vi "TMS Robot_adjust.vi"() -> ()   [LabVIEW 2018]
uses:
  <vilib>/Platform/TimedLoop/XDataNode/timing_clust.ctl
  <vilib>/Platform/TimedLoop/XDataNode/nitl_modes.ctl
  <vilib>/Platform/TimedLoop/XDataNode/wakeup.ctl
  <vilib>/myRIO/Instrument Drivers/Onboard IO/AI/typedefs/AI Reference.ctl
  <vilib>/myRIO/Common/Instrument Driver Framework/Utilities/typedefs/myRIO Generic Hardware Reference.ctl
  <vilib>/myRIO/Common/Instrument Driver Framework/Utilities/typedefs/Hardware Version Enum.ctl
  <vilib>/myRIO/Common/Instrument Driver Framework/Utilities/typedefs/myRIO v1.0 Reference.ctl
  <vilib>/myRIO/Common/Instrument Driver Framework/Utilities/typedefs/Generic FPGA Reference.ctl
  <vilib>/myRIO/Common/Instrument Driver Framework/myRIO v1.0/AI/typedefs/AI Channels List.ctl
  <vilib>/myRIO/Common/Instrument Driver Framework/myRIO v1.0/AI/typedefs/AI Channels Enum.ctl
  <vilib>/myRIO/Common/Instrument Driver Framework/Utilities/typedefs/Analog Scaling Constants List.ctl
  <vilib>/myRIO/Common/Instrument Driver Framework/Utilities/typedefs/Analog Scaling Constants.ctl
  <vilib>/userdefined/High Color/nirio_resource_hc.ctl
  <vilib>/myRIO/Instrument Drivers/Onboard IO/DIO/typedefs/DIO Reference.ctl
  <vilib>/myRIO/Common/Instrument Driver Framework/myRIO v1.0/DIO/typedefs/DIO Channels List.ctl
  <vilib>/myRIO/Common/Instrument Driver Framework/myRIO v1.0/DIO/typedefs/DIO Channels Enum.ctl
  <vilib>/myRIO/Common/Instrument Driver Framework/myRIO v1.0/AI/vis/myRIO v1.1 Open AI.vi
  <vilib>/myRIO/Common/Instrument Driver Framework/myRIO v1.0/DIO/vis/myRIO v1.1 Open DIO.vi
  <vilib>/myRIO/Common/Instrument Driver Framework/Utilities/vis/Validate Channels.vi
  <vilib>/myRIO/Common/Instrument Driver Framework/myRIO v1.0/AI/vis/myRIO v1.0 Reserve AI.vi
  <vilib>/myRIO/Common/Instrument Driver Framework/myRIO v1.0/DIO/vis/myRIO v1.0 Reserve DIO.vi
  <vilib>/myRIO/Common/Instrument Driver Framework/myRIO v1.0/DIO/vis/myRIO v1.0 Close DIO.vi
  <vilib>/myRIO/Common/Instrument Driver Framework/myRIO v1.0/AI/vis/myRIO v1.0 Build MUX Configuration AI.vi
  <vilib>/myRIO/Common/Instrument Driver Framework/myRIO v1.0/Resource Manager/vis/myRIO v1.0 Reserve Channel List.vi
  <vilib>/myRIO/Common/Instrument Driver Framework/myRIO v1.0/DIO/vis/myRIO v1.0 Build MUX Configuration DIO.vi
  <vilib>/myRIO/Common/Instrument Driver Framework/myRIO v1.0/DIO/vis/myRIO v1.0 Unreserve DIO.vi
  <vilib>/myRIO/Common/Instrument Driver Framework/myRIO v1.0/Resource Manager/vis/myRIO v1.0 Reserve Channel.vi
  <vilib>/myRIO/Common/Instrument Driver Framework/myRIO v1.0/Resource Manager/vis/myRIO v1.0 Unreserve Channel.vi
  <vilib>/myRIO/Common/Instrument Driver Framework/myRIO v1.0/Resource Manager/vis/myRIO v1.0 Create Configuration List.vi
  <vilib>/myRIO/Common/Instrument Driver Framework/myRIO v1.0/Resource Manager/vis/myRIO v1.0 Unreserve Channel List.vi
  <vilib>/myRIO/Common/Instrument Driver Framework/myRIO v1.0/Resource Manager/vis/myRIO v1.0 Build Mutex Name.vi
  <vilib>/Utility/VariantDataType/GetNumericInfo.vi
  <vilib>/Utility/error.llb/Error Cluster From Error Code.vi
  <vilib>/myRIO/Common/Instrument Driver Framework/myRIO v1.0/myRIO v1.1 Open.vi
  <vilib>/myRIO/Common/Instrument Driver Framework/Utilities/vis/IO Manager.vi
  <vilib>/myRIO/Common/Instrument Driver Framework/Utilities/vis/Configuration Manager.vi
  <vilib>/myRIO/Common/Instrument Driver Framework/myRIO v1.0/Resource Manager/vis/myRIO v1.0 Configure IO.vi
  <vilib>/myRIO/Common/Instrument Driver Framework/myRIO v1.0/myRIO v1.0 Close.vi
  <vilib>/myRIO/Common/Instrument Driver Framework/myRIO v1.0/AI/vis/myRIO v1.0 Get Scaling Constants AI.vi
  <vilib>/myRIO/Common/Instrument Driver Framework/myRIO v1.0/AI/vis/myRIO v1.0 Read AI.vi
  <vilib>/myRIO/Common/Instrument Driver Framework/myRIO v1.0/DIO/vis/myRIO v1.0 Write DIO.vi
  <vilib>/myRIO/Common/Instrument Driver Framework/myRIO v1.0/DIO/vis/myRIO v1.0 Shutdown DIO.vi
  <vilib>/Platform/TimedLoop/XDataNode/XDataNode.xnode
  <vilib>/myRIO/Instrument Drivers/Onboard IO/DIO/vis/myRIO DIO Open.xnode
  <vilib>/myRIO/Instrument Drivers/Onboard IO/AI/vis/myRIO AI Open.xnode
  <vilib>/Platform/TimedLoop/XDataNode/XDNodeRunTimeDep.lvlib
  <vilib>/myRIO/Instrument Drivers/Onboard IO/DIO/DIO.lvlib
  <vilib>/myRIO/Instrument Drivers/Onboard IO/AI/AI.lvlib
panel:
  out "Phi Real Output  TCP":dbl
  out "Theta Real Output TCP":dbl
  out "Curve Moving TCP":i16
  out "Psi Real Output TCP":dbl
  out "Psi Moving TCP":i16
  out "Z Real Output TCP":dbl
  out "Z Moving TCP":i16
  out "Y Real Output TCP":dbl
  out "Y Moving TCP":i16
  out "X Real Output TCP":dbl
  out "X Moving TCP":i16
  out "Optical R":dbl
  out "Optical L":dbl
  out "Optical psi":dbl
  out "Optical Z":dbl
  out "Optical Y":dbl
  out "Optical X":dbl
  in  "Stop number L":dbl
  in  "Stop number R":dbl
  in  "Stop number x":dbl
  in  "Stop number y":dbl
  in  "Stop number z":dbl
  in  "Stop number psi":dbl
  out "up L":bool
  out "left L":bool
  in  "Step/s  curve":dbl=4.0
  in  "Step difference L":dbl
  in  "Tab Control":enum32{"Azimuth", "Elevation"}(tab)
  in  "Right":bool
  in  "Left":bool
  out "Real Output theta":dbl
  in  "User Input theta":dbl
  in  "Up":bool
  in  "Down":bool
  out "Real Output Phi":dbl
  in  "User Input Phi":dbl=10.45218049
  in  "Motor Input L":dbl
  out "down L":bool
  out "right L":bool
  out "Moving":bool
  out "up R":bool
  out "left R":bool
  in  "Step difference R":dbl
  in  "Motor Input R":dbl
  out "down R":bool
  out "right R":bool
  out "Moving R":bool
  out "up z":bool
  out "down z":bool
  out "right z":bool
  out "left z":bool
  in  "Step/s z":dbl=4.0
  out "Motor Position z":dbl
  in  "User Input z":dbl
  out "Motor State z":dbl
  out "Real Output z":dbl
  in  "Step diff z":dbl
  in  "Up z":bool
  in  "Motor Input z":dbl
  in  "Down z":bool
  out "Moving z":bool
  out "up x":bool
  out "down x":bool
  out "right x":bool
  out "left x":bool
  in  "Step/s x":dbl=4.0
  out "Motor Position x":dbl
  in  "User Input x":dbl
  out "Motor State x":dbl
  out "Real Output x":dbl
  in  "Step diff x":dbl
  in  "Forward x":bool
  in  "Motor Input x":dbl
  in  "Backward x":bool
  out "Moving x":bool
  out "up y":bool
  out "down y":bool
  out "right y":bool
  out "left y":bool
  in  "Step/s y":dbl=4.0
  out "Motor Position y":dbl
  in  "User Input y":dbl
  out "Motor State y":dbl
  out "Real Output y":dbl
  in  "Step diff y":dbl
  in  "Left y":bool
  in  "Motor Input y":dbl
  in  "Right y":bool
  out "Moving y":bool
  out "up psi":bool
  out "down psi":bool
  out "right psi":bool
  out "left psi":bool
  in  "Step/s psi":dbl=4.0
  out "Motor Position psi":dbl
  in  "User Input psi":dbl
  out "Motor State psi":dbl
  out "Real Output psi":dbl
  in  "Step diff psi":dbl
  in  "Left psi":bool
  in  "Motor Input psi":dbl
  in  "Right psi":bool
  out "Moving psi":bool
  in  "Stop":bool
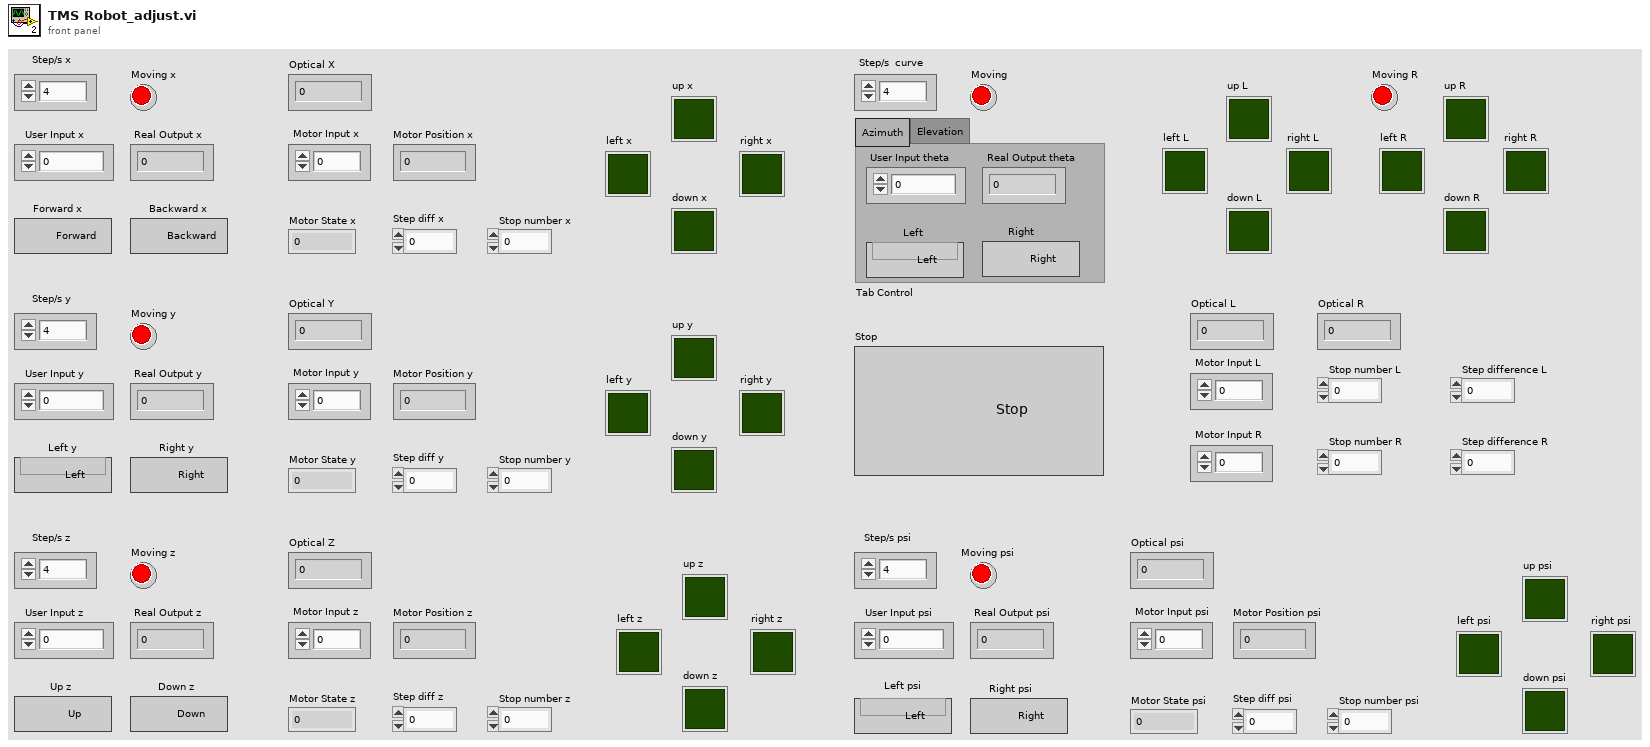
[diagram p1: front panel]
types:
  T1 = enum16{"big-endian, network order", "native, host order", "little-endian"}
  T2 = typedef "nirio_resource_hc.ctl" = tag
  T3 = typedef "Hardware Version Enum.ctl" = enum16{"Unknown", "myRIO-1900", "myRIO-1950", "roboRIO", "NI ELVIS RIO CM", "ELVIS III"}
  T4 = typedef "XDNodeRunTimeDep.lvlib/timing_clust.ctl" = cluster{"Expected End [f-1]":u64, "Actual End [f-1]":u64, "Finished Late? [f-1]":bool, "Expected End [i-1]":u64, "Actual End [i-1]":u64, "Finished Late? [i-1]":bool, "Expected Start [i]":u64, "Actual Start [i]":u64, "Expected Start [f]":u64, "Actual Start [f]":u64, "Source Name":string, "Structure Name":string, "Period":i64, "Deadline":i64, "Offset":i64, "Start":i64, "Priority":i32, "Timeout":i32, "Mode":T5, "Wakeup Reason":T6, "Error":errorcluster, "Source Type":string, "Secondary Source Type":string, "Global End Time":u64, "Global Start Time":u64, "Frame Duration":u64, "Iteration Duration":u64, "Assigned CPU":i32, "I/O Scan Engine Mode":u32}
  T5 = typedef "XDNodeRunTimeDep.lvlib/nitl_modes.ctl" = enum32{"No Change", "Process missed periods, maintain original phase", "Discard missed periods, maintain original phase", "Process missed periods, ignore original phase", "Discard missed periods, ignore original phase"}
  T6 = typedef "XDNodeRunTimeDep.lvlib/wakeup.ctl" = enum32{"Normal", "Aborted", "Asynchronous wakeup", "Timing source error", "Timed loop error", "Timeout"}
  T7 = typedef "AI.lvlib/AI Reference.ctl" = cluster{"myRIO Reference":T8, "AI Channels List":T11, "AI Scaling Constants List":T13}
  T8 = typedef "myRIO Generic Hardware Reference.ctl" = cluster{"myRIO Model":T3, "myRIO Hardware Reference":T9}
  T9 = typedef "myRIO v1.0 Reference.ctl" = cluster{"Generic FPGA Reference":T10, "Allow multiple opens":bool}
  T10 = typedef "Generic FPGA Reference.ctl" = refnum<k20>
  T11 = typedef "AI Channels List.ctl" = T12[]
  T12 = typedef "AI Channels Enum.ctl" = enum16{"Not Connected", "AudioIn/Left", "AudioIn/Right", "C/AI0", "C/AI1", "A/AI0", "A/AI1", "A/AI2", "A/AI3", "A/AI4", "A/AI5", "A/AI6", "A/AI7", "B/AI0", "B/AI1", "B/AI2", "B/AI3", "B/AI4", "B/AI5", "B/AI6", "B/AI7", "AI/AI0", "AI/AI1", "AI/AI2", "AI/AI3", "A/AI0 (DIFF)", "A/AI1 (DIFF)", "A/AI2 (DIFF)", "A/AI3 (DIFF)", "B/AI0 (DIFF)", "B/AI1 (DIFF)", "B/AI2 (DIFF)", "B/AI3 (DIFF)"}
  T13 = typedef "Analog Scaling Constants List.ctl" = T14[]
  T14 = typedef "Analog Scaling Constants.ctl" = cluster{"LSB Weight (Volts)":dbl, "Offset (Volts)":dbl, "Signed?":bool}
  T15 = typedef "DIO.lvlib/DIO Reference.ctl" = cluster{"myRIO Reference":T8, "DIO Channels List":T16}
  T16 = typedef "DIO Channels List.ctl" = T17[]
  T17 = typedef "DIO Channels Enum.ctl" = enum16{"Not Connected", "C/DIO0", "C/DIO1", "C/DIO2", "C/DIO3", "C/DIO4", "C/DIO5", "C/DIO6", "C/DIO7", "A/DIO0", "A/DIO1", "A/DIO2", "A/DIO3", "A/DIO4", "A/DIO5", "A/DIO6", "A/DIO7", "A/DIO8", "A/DIO9", "A/DIO10", "A/DIO11", "A/DIO12", "A/DIO13", "A/DIO14", "A/DIO15", "A/DIO16", "A/DIO17", "A/DIO18", "A/DIO19", "B/DIO0", "B/DIO1", "B/DIO2", "B/DIO3", "B/DIO4", "B/DIO5", "B/DIO6", "B/DIO7", "B/DIO8", "B/DIO9", "B/DIO10", "B/DIO11", "B/DIO12", "B/DIO13", "B/DIO14", "B/DIO15", "B/DIO16", "B/DIO17", "B/DIO18", "B/DIO19", "LED0", "LED1", "LED2", "LED3", "Button0", "DIO/DIO0", "DIO/DIO1", "DIO/DIO2", "DIO/DIO3", "DIO/DIO4", "DIO/DIO5", "DIO/DIO6", "DIO/DIO7", "DIO/DIO8", "DIO/DIO9", "SPI/CS0", "SPI/CS1", "SPI/CS2", "SPI/CS3", "LED RADIO (Green)", "LED RADIO (Red)", "LED COMM (Green)", "LED COMM (Red)", "LED MODE (Green)", "LED MODE (Red)"}
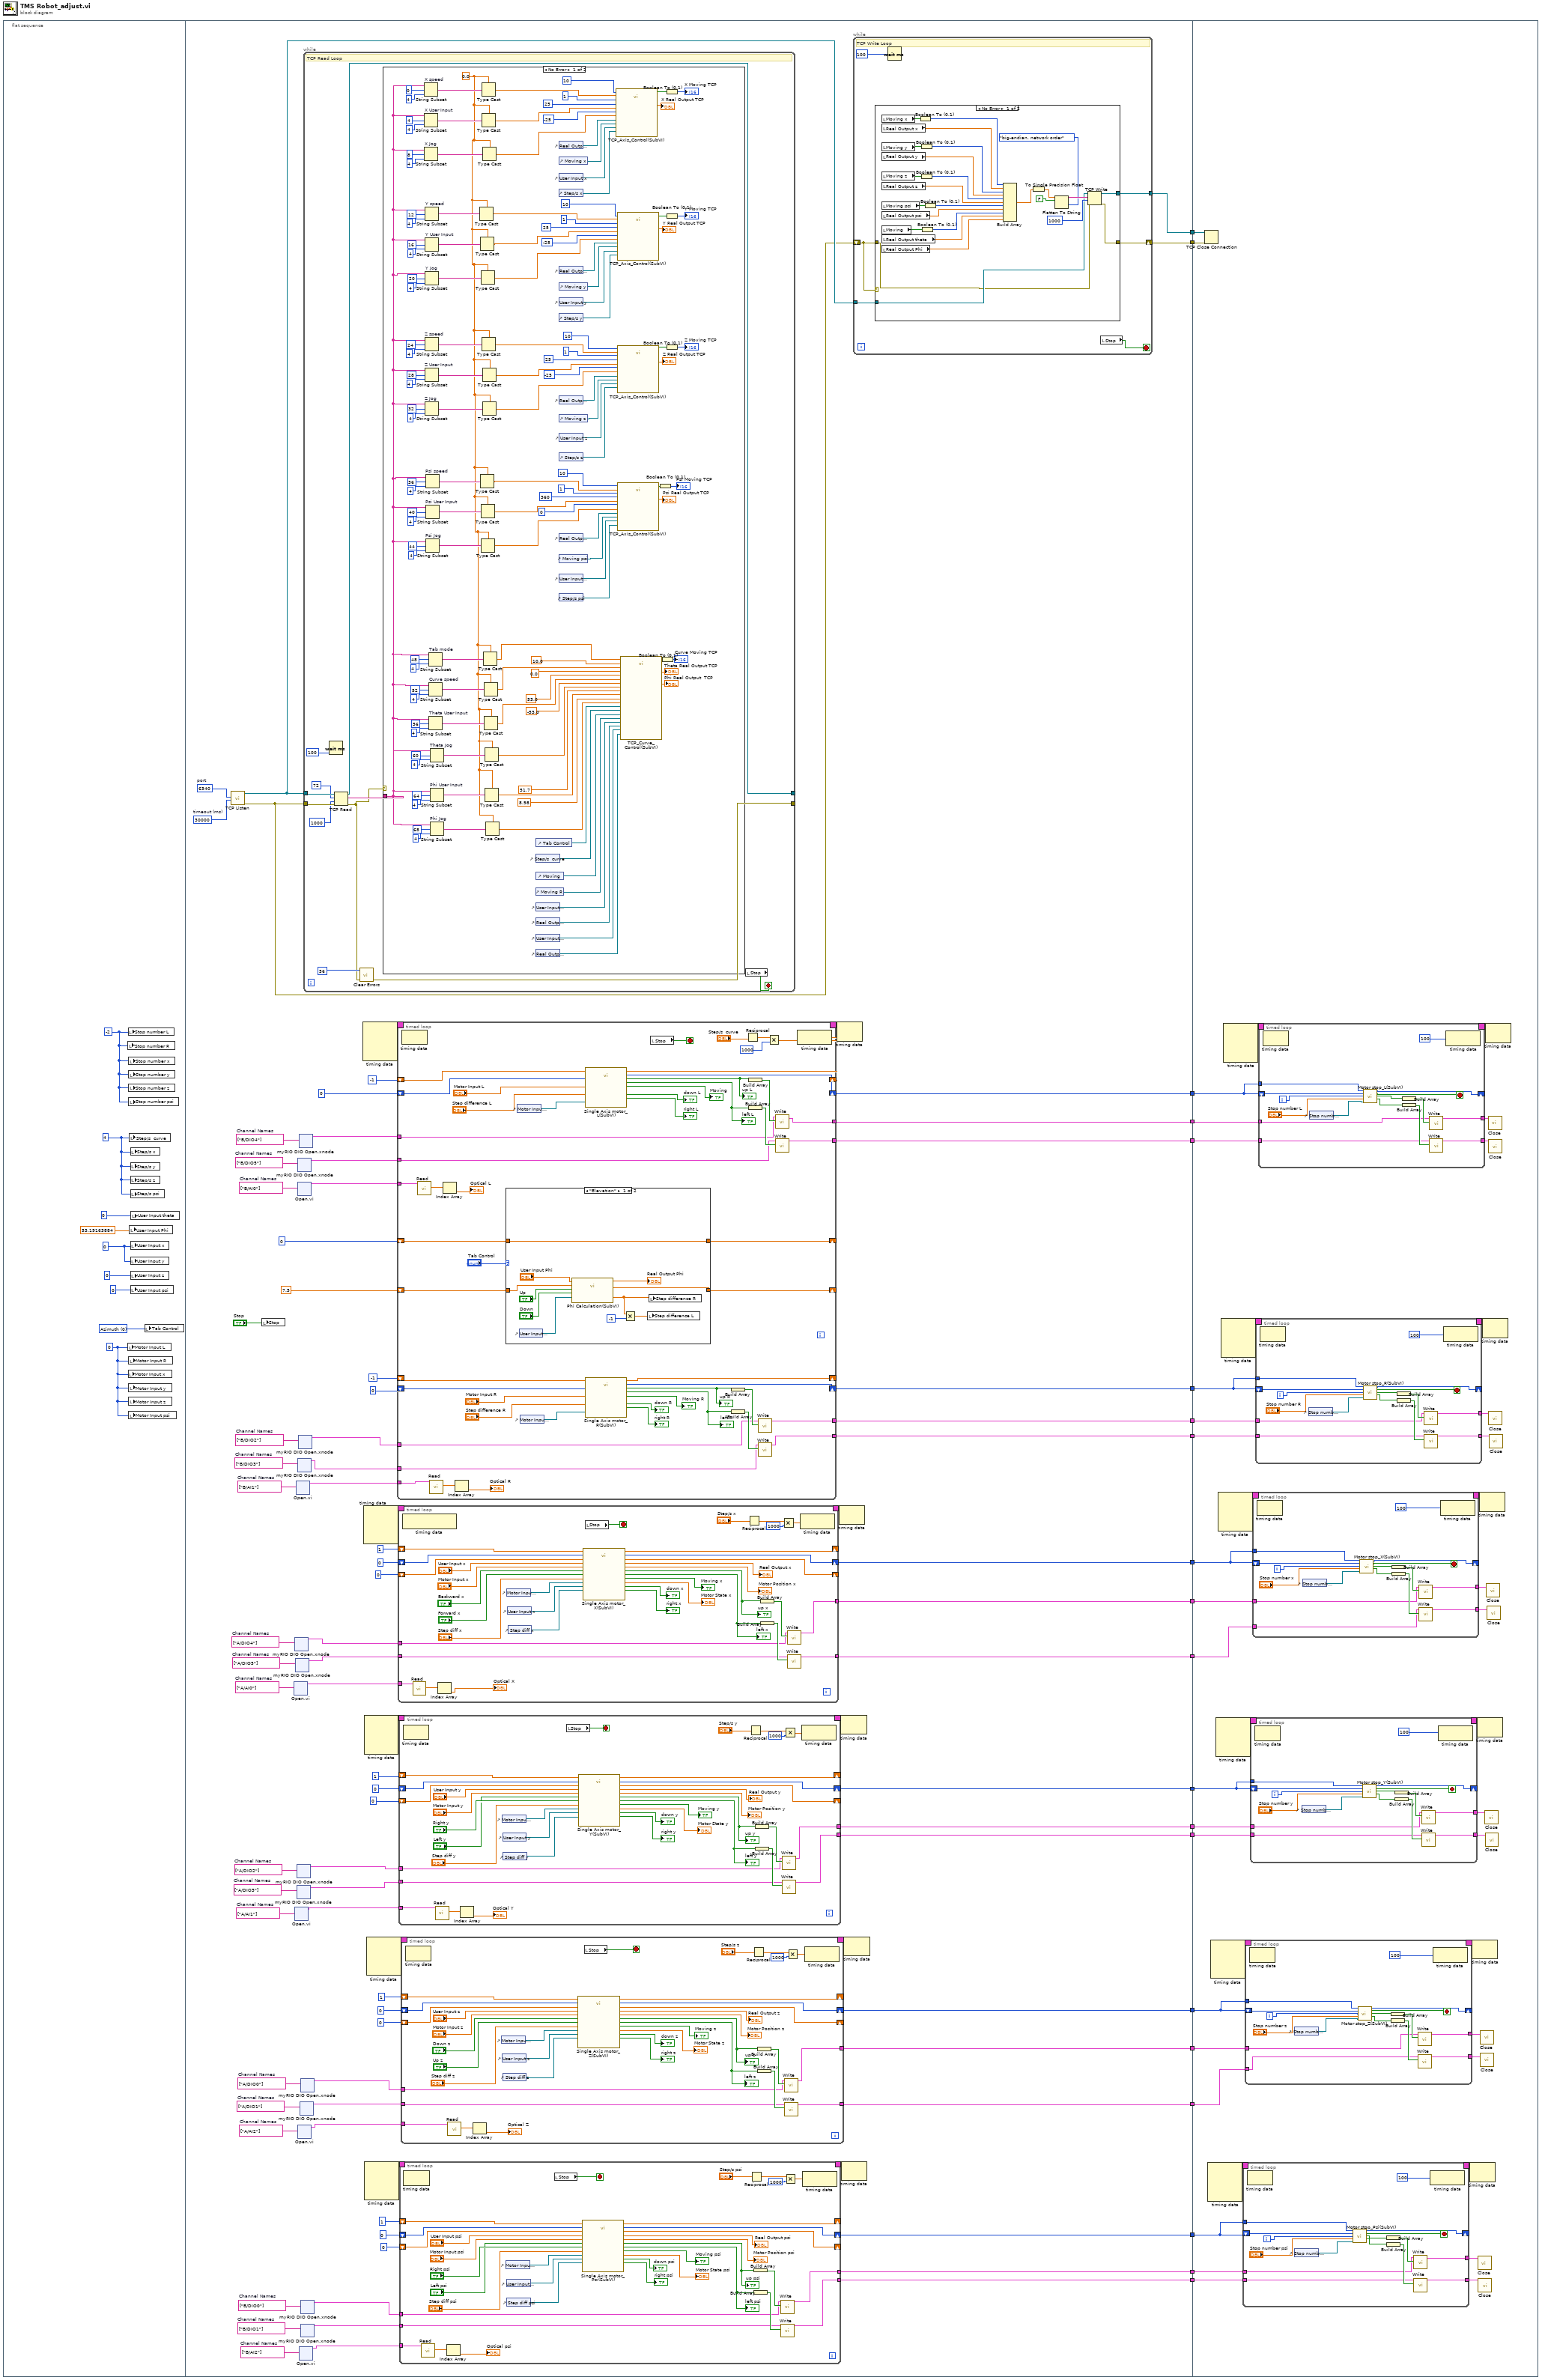
[diagram p0: block diagram]
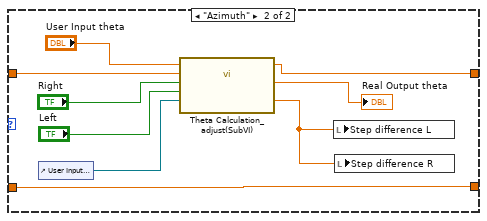
[diagram p4: hidden frame]
diagram:
  n1 = flat-sequence {
    tunnel: [w96] -> w20
    tunnel: [w95] -> w19
    tunnel: [w94] -> w18
    tunnel: [w93] -> w17
    tunnel: [w92] -> w16
    tunnel: [w91] -> w15
    tunnel: [w90] -> w14
    tunnel: [w89] -> w13
    tunnel: [w88] -> w12
    tunnel: [w87] -> w11
    tunnel: [w86] -> w10
    tunnel: [w85] -> w9
    tunnel: [w84] -> w8
    tunnel: [w83] -> w7
    tunnel: [w82] -> w6
    tunnel: [w81] -> w5
    tunnel: [w80] -> w4
    tunnel: [w79] -> w3
    tunnel: [w33] -> w2
    tunnel: [w32] -> w1
    tunnel: w20 -> [w887]
    tunnel: w19 -> [w884]
    tunnel: w18 -> [w881]
    tunnel: w17 -> [w878]
    tunnel: w16 -> [w875]
    tunnel: w15 -> [w872]
    tunnel: w14 -> [w869]
    tunnel: w13 -> [w868]
    tunnel: w12 -> [w867]
    tunnel: w11 -> [w866]
    tunnel: w10 -> [w861]
    tunnel: w9 -> [w860]
    tunnel: w8 -> [w859]
    tunnel: w7 -> [w858]
    tunnel: w6 -> [w857]
    tunnel: w5 -> [w856]
    tunnel: w4 -> [w855]
    tunnel: w3 -> [w854]
    tunnel: w2 -> [w847]
    tunnel: w1 -> [w846]
    frame #0 {
      w21 = 0
      w22 = u16 0 items=["Azimuth"]
      w24 = 0
      w28 = -2
      w27 = 4
      n2 = local write "Stop number R"(w28) -> ()
      n3 = local write "Motor Input L"(w21) -> ()
      n4 = local write "Stop number L"(w28) -> ()
      n5 = local write "Motor Input x"(w21) -> ()
      n6 = local write "Stop number x"(w28) -> ()
      n7 = local write "Stop number y"(w28) -> ()
      n8 = local write "Stop number z"(w28) -> ()
      n9 = local write "Stop number psi"(w28) -> ()
      n10 = local write "Motor Input R"(w21) -> ()
      n11 = local write "Motor Input y"(w21) -> ()
      n12 = local write "Motor Input z"(w21) -> ()
      n13 = local write "Motor Input psi"(w21) -> ()
      n14 = local write "Step/s  curve"(w27) -> ()
      n15 = local write "User Input Phi"(53.19163884) -> ()
      n16 = local write "Step/s x"(w27) -> ()
      n17 = local write "Step/s y"(w27) -> ()
      n18 = local write "Step/s z"(w27) -> ()
      n19 = local write "Step/s psi"(w27) -> ()
      n20 = local write "User Input x"(w24) -> ()
      n21 = local write "User Input y"(w24) -> ()
      n22 = local write "User Input z"(0) -> ()
      n23 = local write "User Input psi"(0) -> ()
      n24 = local write "User Input theta"(0) -> ()
      n25 = local write "Tab Control"(w22) -> ()
    }
    frame #1 {
      w34 = u16 6340  # port
      w35 = 30000  # timeout (ms)
      w44 = tag[] ["B/AI0"]  # Channel Names
      w46 = tag[] ["B/AI1"]  # Channel Names
      w49 = tag[] ["B/AI2"]  # Channel Names
      w51 = tag[] ["A/AI2"]  # Channel Names
      w53 = tag[] ["A/AI1"]  # Channel Names
      w55 = tag[] ["A/AI0"]  # Channel Names
      w59 = tag[] ["B/DIO1"]  # Channel Names
      w58 = tag[] ["B/DIO0"]  # Channel Names
      w63 = tag[] ["A/DIO1"]  # Channel Names
      w62 = tag[] ["A/DIO0"]  # Channel Names
      w67 = tag[] ["A/DIO3"]  # Channel Names
      w66 = tag[] ["A/DIO2"]  # Channel Names
      w71 = tag[] ["A/DIO5"]  # Channel Names
      w70 = tag[] ["A/DIO4"]  # Channel Names
      w75 = tag[] ["B/DIO5"]  # Channel Names
      w74 = tag[] ["B/DIO4"]  # Channel Names
      w78 = tag[] ["B/DIO3"]  # Channel Names
      w77 = tag[] ["B/DIO2"]  # Channel Names
      n26 = call <vilib>:"TCP Listen.vi"("timeout ms (wait forever: -1)"=w35, "port"=w34) -> ("error out"=w30:errorcluster, "connection ID"=w31:refnum<k5>)  [unwired: 5 in, 3 out]
      n27 = local write "Stop"("Stop") -> ()
      n28 = xnode "Open.vi"("Channel Names"=w55) -> ("AI Ref Out"=w54:T7)  [unwired: 2 in, 1 out]
      n29 = xnode "myRIO DIO Open.xnode"("Channel Names"=w70) -> ("DIO Ref Out"=w69:T15)  [unwired: 2 in, 1 out]
      n30 = xnode "Open.vi"("Channel Names"=w53) -> ("AI Ref Out"=w52:T7)  [unwired: 2 in, 1 out]
      n31 = xnode "myRIO DIO Open.xnode"("Channel Names"=w71) -> ("DIO Ref Out"=w68:T15)  [unwired: 2 in, 1 out]
      n32 = xnode "Open.vi"("Channel Names"=w46) -> ("AI Ref Out"=w45:T7)  [unwired: 2 in, 1 out]
      n33 = xnode "myRIO DIO Open.xnode"("Channel Names"=w67) -> ("DIO Ref Out"=w64:T15)  [unwired: 2 in, 1 out]
      n34 = xnode "myRIO DIO Open.xnode"("Channel Names"=w66) -> ("DIO Ref Out"=w65:T15)  [unwired: 2 in, 1 out]
      n35 = xnode "myRIO DIO Open.xnode"("Channel Names"=w75) -> ("DIO Ref Out"=w72:T15)  [unwired: 2 in, 1 out]
      n36 = xnode "Open.vi"("Channel Names"=w44) -> ("AI Ref Out"=w43:T7)  [unwired: 2 in, 1 out]
      n37 = xnode "myRIO DIO Open.xnode"("Channel Names"=w78) -> ("DIO Ref Out"=w47:T15)  [unwired: 2 in, 1 out]
      n38 = xnode "Open.vi"("Channel Names"=w51) -> ("AI Ref Out"=w50:T7)  [unwired: 2 in, 1 out]
      n39 = xnode "myRIO DIO Open.xnode"("Channel Names"=w77) -> ("DIO Ref Out"=w76:T15)  [unwired: 2 in, 1 out]
      n40 = xnode "myRIO DIO Open.xnode"("Channel Names"=w74) -> ("DIO Ref Out"=w73:T15)  [unwired: 2 in, 1 out]
      n41 = xnode "Open.vi"("Channel Names"=w49) -> ("AI Ref Out"=w48:T7)  [unwired: 2 in, 1 out]
      n42 = xnode "myRIO DIO Open.xnode"("Channel Names"=w63) -> ("DIO Ref Out"=w60:T15)  [unwired: 2 in, 1 out]
      n43 = xnode "myRIO DIO Open.xnode"("Channel Names"=w62) -> ("DIO Ref Out"=w61:T15)  [unwired: 2 in, 1 out]
      n44 = xnode "myRIO DIO Open.xnode"("Channel Names"=w59) -> ("DIO Ref Out"=w56:T15)  [unwired: 2 in, 1 out]
      n45 = xnode "myRIO DIO Open.xnode"("Channel Names"=w58) -> ("DIO Ref Out"=w57:T15)  [unwired: 2 in, 1 out]
      n46 = while {
        tunnel: [w153] -> _
        tunnel: w31 -> [w162]
        tunnel: w30 -> [w163]
        tunnel: [w154] -> _
        stop <- w156 stop-if-true
        # "TCP Read Loop"
        n47 = Wait (ms)(milliseconds to wait=100) -> ()  [unwired: 1 out]
        n48 = TCP Read(connection ID=w162, bytes to read=72, error in (no error)=w163, 9:1000 ("timeout ms (25000)")) -> (connection ID out=w154:refnum<k5>, data out=w158:string, error out=w155:errorcluster)  [unwired: 1 out]
        n49 = call <vilib>:"Clear Errors.vi"("error in (no error)"=w155, "specific error code to clear (0: all)"=56) -> ("error out"=w153:errorcluster)  [unwired: 4 in, 1 out]
        n50 = case shown="No Error" w155 {
          tunnel: w158 -> [w197 _]
          frame No Error {
            w196 = sgl 0.0 ("x")
            n51 = String Subset "X speed"(string=w197, offset (0)=0, length (rest)=4) -> (substring=w289:string)
            n52 = String Subset "X User Input"(string=w197, offset (0)=4, length (rest)=4) -> (substring=w285:string)
            n53 = String Subset "X Jog"(string=w197, offset (0)=8, length (rest)=4) -> (substring=w281:string)
            n54 = String Subset "Z speed"(string=w197, offset (0)=24, length (rest)=4) -> (substring=w257:string)
            n55 = String Subset "Z User Input"(string=w197, offset (0)=28, length (rest)=4) -> (substring=w254:string)
            n56 = String Subset "Z Jog"(string=w197, offset (0)=32, length (rest)=4) -> (substring=w251:string)
            n57 = String Subset "Y speed"(string=w197, offset (0)=12, length (rest)=4) -> (substring=w272:string)
            n58 = String Subset "Y User Input"(string=w197, offset (0)=16, length (rest)=4) -> (substring=w273:string)
            n59 = String Subset "Y Jog"(string=w197, offset (0)=20, length (rest)=4) -> (substring=w271:string)
            n60 = String Subset "Psi speed"(string=w197, offset (0)=36, length (rest)=4) -> (substring=w243:string)
            n61 = String Subset "Psi User Input"(string=w197, offset (0)=40, length (rest)=4) -> (substring=w244:string)
            n62 = String Subset "Psi Jog"(string=w197, offset (0)=44, length (rest)=4) -> (substring=w242:string)
            n63 = String Subset "Tab mode"(string=w197, offset (0)=48, length (rest)=4) -> (substring=w208:string)
            n64 = String Subset "Curve speed"(string=w197, offset (0)=52, length (rest)=4) -> (substring=w209:string)
            n65 = String Subset "Theta User Input"(string=w197, offset (0)=56, length (rest)=4) -> (substring=w207:string)
            n66 = String Subset "Theta Jog"(string=w197, offset (0)=60, length (rest)=4) -> (substring=w199:string)
            n67 = String Subset "Phi User Input"(string=w197, offset (0)=64, length (rest)=4) -> (substring=w200:string)
            n68 = String Subset "Phi Jog"(string=w197, offset (0)=68, length (rest)=4) -> (substring=w198:string)
            n69 = Type Cast(type=w196, x=w272) -> (*(type *) &x=w270:sgl)
            n70 = Type Cast(type=w196, x=w273) -> (*(type *) &x=w265:sgl)
            n71 = Type Cast(type=w196, x=w243) -> (*(type *) &x=w229:sgl)
            n72 = Type Cast(type=w196, x=w271) -> (*(type *) &x=w264:sgl)
            n73 = Type Cast(type=w196, x=w244) -> (*(type *) &x=w226:sgl)
            n74 = Type Cast(type=w196, x=w242) -> (*(type *) &x=w224:sgl)
            n75 = Type Cast(type=w196, x=w289) -> (*(type *) &x=w288:sgl)
            n76 = Type Cast(type=w196, x=w285) -> (*(type *) &x=w284:sgl)
            n77 = Type Cast(type=w196, x=w257) -> (*(type *) &x=w241:sgl)
            n78 = Type Cast(type=w196, x=w281) -> (*(type *) &x=w280:sgl)
            n79 = Type Cast(type=w196, x=w254) -> (*(type *) &x=w237:sgl)
            n80 = Type Cast(type=w196, x=w251) -> (*(type *) &x=w235:sgl)
            n81 = Type Cast(type=w196, x=w208) -> (*(type *) &x=w195:sgl)
            n82 = Type Cast(type=w196, x=w209) -> (*(type *) &x=w194:sgl)
            n83 = Type Cast(type=w196, x=w207) -> (*(type *) &x=w193:sgl)
            n84 = Type Cast(type=w196, x=w199) -> (*(type *) &x=w188:sgl)
            n85 = Type Cast(type=w196, x=w200) -> (*(type *) &x=w187:sgl)
            n86 = Type Cast(type=w196, x=w198) -> (*(type *) &x=w186:sgl)
            n87 = control-ref of="Tab Control"() -> (w183:refnum<vi>)
            n88 = control-ref of="Step/s  curve"() -> (w182:refnum<vi>)
            n89 = control-ref of="Moving"() -> (w181:refnum<vi>)
            n90 = control-ref of="Moving R"() -> (w180:refnum<vi>)
            n91 = control-ref of="User Input theta"() -> (w179:refnum<vi>)
            n92 = control-ref of="Real Output theta"() -> (w178:refnum<vi>)
            n93 = control-ref of="User Input Phi"() -> (w177:refnum<vi>)
            n94 = control-ref of="Real Output Phi"() -> (w176:refnum<vi>)
            n95 = control-ref of="Real Output x"() -> (w296:refnum<vi>)
            n96 = control-ref of="Moving x"() -> (w297:refnum<vi>)
            n97 = control-ref of="User Input x"() -> (w298:refnum<vi>)
            n98 = control-ref of="Step/s x"() -> (w299:refnum<vi>)
            n99 = control-ref of="Real Output y"() -> (w263:refnum<vi>)
            n100 = control-ref of="Moving y"() -> (w262:refnum<vi>)
            n101 = control-ref of="User Input y"() -> (w261:refnum<vi>)
            n102 = control-ref of="Step/s y"() -> (w260:refnum<vi>)
            n103 = control-ref of="Real Output z"() -> (w234:refnum<vi>)
            n104 = control-ref of="Moving z"() -> (w233:refnum<vi>)
            n105 = control-ref of="User Input z"() -> (w232:refnum<vi>)
            n106 = control-ref of="Step/s z"() -> (w231:refnum<vi>)
            n107 = control-ref of="Real Output psi"() -> (w223:refnum<vi>)
            n108 = control-ref of="Moving psi"() -> (w222:refnum<vi>)
            n109 = control-ref of="User Input psi"() -> (w221:refnum<vi>)
            n110 = control-ref of="Step/s psi"() -> (w220:refnum<vi>)
            n111 = call "TCP_Axis_Control(SubVI).vi"("Speed Max"=10, "Step/s"=w288, "Speed Mini"=1, "Position Max"=25, "User Input"=w284, "Position Mini"=-25, "Jog"=w280, "Step/s Ref"=w299, "User Input Ref"=w298, "Moving Ref"=w297, "Real Output Ref"=w296) -> ("Moving"=w216:bool, "Real Output"=→"X Real Output TCP":dbl)  [unwired: 13 in, 2 out]
            n112 = call "TCP_Axis_Control(SubVI).vi"("Speed Max"=10, "Step/s"=w270, "Speed Mini"=1, "Position Max"=25, "User Input"=w265, "Position Mini"=-25, "Jog"=w264, "Step/s Ref"=w260, "User Input Ref"=w261, "Moving Ref"=w262, "Real Output Ref"=w263) -> ("Moving"=w217:bool, "Real Output"=→"Y Real Output TCP":dbl)  [unwired: 13 in, 2 out]
            n113 = call "TCP_Axis_Control(SubVI).vi"("Speed Max"=10, "Step/s"=w241, "Speed Mini"=1, "Position Max"=25, "User Input"=w237, "Position Mini"=-25, "Jog"=w235, "Step/s Ref"=w231, "User Input Ref"=w232, "Moving Ref"=w233, "Real Output Ref"=w234) -> ("Moving"=w218:bool, "Real Output"=→"Z Real Output TCP":dbl)  [unwired: 13 in, 2 out]
            n114 = call "TCP_Axis_Control(SubVI).vi"("Speed Max"=10, "Step/s"=w229, "Speed Mini"=1, "Position Max"=360, "User Input"=w226, "Position Mini"=0, "Jog"=w224, "Step/s Ref"=w220, "User Input Ref"=w221, "Moving Ref"=w222, "Real Output Ref"=w223) -> ("Moving"=w219:bool, "Real Output"=→"Psi Real Output TCP":dbl)  [unwired: 13 in, 2 out]
            n115 = call "TCP_Curve_Control(SubVI).vi"("Tab mode"=w195, "Speed Max"=10.0, "Step/s"=w194, "Speed Mini"=0.0, "Theta Max"=53.0, "User Input Theta"=w193, "Theta Mini"=-53.0, "Jog Theta"=w188, "Real Output Phi Ref"=w176, "Phi Max"=51.7, "User Input Phi Ref"=w177, "User Input Phi"=w187, "Real Output Theta Ref"=w178, "Phi Mini"=8.98, "User Input Theta Ref"=w179, "Jog Phi"=w186, "Moving R Ref"=w180, "Tab Control Ref"=w183, "Moving L Ref"=w181, "Step/s Ref"=w182) -> ("Moving"=w175:bool, "Real Output Theta"=→"Theta Real Output TCP":dbl, "Real Output  Phi"=→"Phi Real Output  TCP":dbl)  [unwired: 1 in, 4 out]
            n116 = Boolean To (0,1)(Boolean=w219) -> (0, 1=→"Psi Moving TCP":i16)
            n117 = Boolean To (0,1)(Boolean=w175) -> (0, 1=→"Curve Moving TCP":i16)
            n118 = Boolean To (0,1)(Boolean=w216) -> (0, 1=→"X Moving TCP":i16)
            n119 = Boolean To (0,1)(Boolean=w217) -> (0, 1=→"Y Moving TCP":i16)
            n120 = Boolean To (0,1)(Boolean=w218) -> (0, 1=→"Z Moving TCP":i16)
          }
          frame Error {
          }
        }
        n121 = local read "Stop"() -> (w156:bool)
      }
      n122 = node-c288() -> (w118:T4)  [unwired: 4 in]
      n123 = node-c288() -> (w111:T4)  [unwired: 4 in]
      n124 = node-c288() -> (w109:T4)  [unwired: 4 in]
      n125 = node-c288() -> (w101:T4)  [unwired: 4 in]
      n126 = node-c288() -> (w113:T4)  [unwired: 4 in]
      n127 = timed-loop {
        shift-right: [w807] -> w96
        shift-left: 0 -> [w808]
        shift-right: [w809] -> _
        shift-left: -1 -> [w810]
        shift-right: [w814] -> _
        shift-left: 0 -> [w815]
        timing: w118 -> [_]
        timing-out: [_] -> w117
        shift-right: [w812] -> _
        shift-left: 7.5 -> [w811]
        shift-right: [w796] -> w95
        shift-left: 0 -> [w797]
        shift-right: [w794] -> _
        shift-left: -1 -> [w795]
        tunnel: w76 -> [w785]
        tunnel: w47 -> [w784]
        tunnel: w72 -> [w779]
        tunnel: w73 -> [w778]
        tunnel: [w777] -> w90
        tunnel: [w776] -> w89
        tunnel: [w775] -> w88
        tunnel: [w774] -> w87
        tunnel: w45 -> [w772]
        tunnel: w43 -> [w770]
        stop <- w802 stop-if-true
        n128 = node-c288() -> ()  [unwired: 1 in, 1 out]
        n129 = call <vilib>:"Read.vi"("AI Ref In"=w770) -> ("Values"=w771:dbl[])  [unwired: 8 in, 2 out]
        n130 = call <vilib>:"Read.vi"("AI Ref In"=w772) -> ("Values"=w773:dbl[])  [unwired: 8 in, 2 out]
        n131 = Index Array(array=w771) -> (element=→"Optical L":dbl)  [unwired: 1 in]
        n132 = Index Array(array=w773) -> (element=→"Optical R":dbl)  [unwired: 1 in]
        n133 = case shown="\"Elevation\"" "Tab Control" {
          tunnel: w811 -> [w829 w839]
          tunnel: [w828 w839] -> w812
          tunnel: w815 -> [w830 w836]
          tunnel: [w830 w835] -> w814
          frame "Elevation" {
            n134 = control-ref of="User Input Phi"() -> (w823:refnum<vi>)
            n135 = call "Phi Calculation(SubVI).vi"(0:"User Input Phi"="User Input Phi", "Position=0, I"=w829, "Up"="Up", "Down"="Down", 11:"User Input Phi"=w823) -> ("Real output phi"=→"Real Output Phi":dbl, "Position=0, O"=w828:dbl, "Step diff"=w820:dbl)  [unwired: 8 in]
            n136 = Multiply(x=w820, y=-1) -> (x*y=w821:dbl)
            n137 = local write "Step difference L"(w821) -> ()
            n138 = local write "Step difference R"(w820) -> ()
          }
          frame "Azimuth" {
            n139 = control-ref of="User Input theta"() -> (w837:refnum<vi>)
            n140 = call "Theta Calculation_adjust(SubVI).vi"(0:"User Input theta"="User Input theta", "Position=-85, I"=w836, "Right"="Right", "Left"="Left", 11:"User Input theta"=w837) -> ("Position=-85, O"=w835:dbl, "Real output theta"=→"Real Output theta":dbl, "Step diff"=w833:dbl)  [unwired: 8 in]
            n141 = local write "Step difference L"(w833) -> ()
            n142 = local write "Step difference R"(w833) -> ()
          }
        }
        n143 = control-ref of="Motor Input L"() -> (w804:refnum<vi>)
        n144 = control-ref of="Motor Input R"() -> (w799:refnum<vi>)
        n145 = call "Single Axis motor_R(SubVI).vi"("State=1, I"=w795, "Motor=0, I"=w797, "Motor Input"="Motor Input R", "Step diff"="Step difference R", "Motor Input_L"=w799) -> ("right"=→"right R":bool, "State=1, O"=w794:dbl, "Motor=0, O"=w796:i32, "up"=w787:bool, "left"=w786:bool, "Moving"=→"Moving R":bool, "down"=→"down R":bool)  [unwired: 14 in, 2 out]
        "up R" <- w787
        "left R" <- w786
        n146 = call "Single Axis motor_L(SubVI).vi"("State=1, I"=w810, "Motor=0, I"=w808, "Motor Input"="Motor Input L", "Step diff"="Step difference L", "Motor Input_L"=w804) -> ("right"=→"right L":bool, "State=1, O"=w809:dbl, "Motor=0, O"=w807:i32, "up"=w781:bool, "left"=w780:bool, "Moving"=→"Moving":bool, "down"=→"down L":bool)  [unwired: 14 in, 2 out]
        "up L" <- w781
        "left L" <- w780
        n147 = local read "Stop"() -> (w802:bool)
        n148 = Build Array(w787) -> (w789:bool[])
        n149 = Build Array(w786) -> (w788:bool[])
        n150 = Reciprocal(x="Step/s  curve") -> (1/x=w818:dbl)
        n151 = Build Array(w781) -> (w783:bool[])
        n152 = Build Array(w780) -> (w782:bool[])
        n153 = call <vilib>:"Write.vi"("Values"=w789, "DIO Ref In"=w785) -> ("DIO Ref Out"=w775:T15)  [unwired: 7 in, 1 out]
        n154 = call <vilib>:"Write.vi"("Values"=w788, "DIO Ref In"=w784) -> ("DIO Ref Out"=w774:T15)  [unwired: 7 in, 1 out]
        n155 = Multiply(x=w818, y=1000) -> (x*y=w816:dbl)
        n156 = call <vilib>:"Write.vi"("Values"=w783, "DIO Ref In"=w778) -> ("DIO Ref Out"=w777:T15)  [unwired: 7 in, 1 out]
        n157 = call <vilib>:"Write.vi"("Values"=w782, "DIO Ref In"=w779) -> ("DIO Ref Out"=w776:T15)  [unwired: 7 in, 1 out]
        n158 = node-c288(w816) -> ()  [unwired: 1 out]
      }
      n159 = timed-loop {
        shift-right: [w703] -> w94
        shift-left: 0 -> [w714]
        shift-right: [w704] -> _
        shift-left: 1 -> [w715]
        shift-right: [w699] -> _
        shift-left: 0 -> [w713]
        timing: w111 -> [_]
        timing-out: [_] -> w110
        tunnel: w69 -> [w690]
        tunnel: w68 -> [w689]
        tunnel: [w688] -> w86
        tunnel: [w687] -> w85
        tunnel: w54 -> [w685]
        stop <- w697 stop-if-true
        n160 = node-c288() -> ()  [unwired: 1 in, 1 out]
        n161 = call <vilib>:"Read.vi"("AI Ref In"=w685) -> ("Values"=w686:dbl[])  [unwired: 8 in, 2 out]
        n162 = Index Array(array=w686) -> (element=→"Optical X":dbl)  [unwired: 1 in]
        n163 = control-ref of="Motor Input x"() -> (w707:refnum<vi>)
        n164 = control-ref of="User Input x"() -> (w706:refnum<vi>)
        n165 = control-ref of="Step diff x"() -> (w705:refnum<vi>)
        n166 = call "Single Axis motor_X(SubVI).vi"("State=1, I"=w715, "Motor=0, I"=w714, "Position=0, I"=w713, "User Input"="User Input x", "Motor Input"="Motor Input x", "Backward"="Backward x", "Forward"="Forward x", "Step diff"="Step diff x", "Motor input_L"=w707, "User input_L"=w706, "Step diff_L"=w705) -> ("right"=→"right x":bool, "down"=→"down x":bool, "Motor State"=→"Motor State x":dbl, "State=1, O"=w704:dbl, "Motor=0, O"=w703:i32, "Position=0, O"=w699:dbl, "Real Output"=→"Real Output x":dbl, "Motor Position"=→"Motor Position x":dbl, "up"=w692:bool, "left"=w691:bool, "Moving"=→"Moving x":bool)  [unwired: 5 in, 1 out]
        "up x" <- w692
        "left x" <- w691
        n167 = local read "Stop"() -> (w697:bool)
        n168 = Reciprocal(x="Step/s x") -> (1/x=w718:dbl)
        n169 = Build Array(w692) -> (w694:bool[])
        n170 = Build Array(w691) -> (w693:bool[])
        n171 = Multiply(x=w718, y=1000) -> (x*y=w716:dbl)
        n172 = call <vilib>:"Write.vi"("Values"=w694, "DIO Ref In"=w690) -> ("DIO Ref Out"=w687:T15)  [unwired: 7 in, 1 out]
        n173 = call <vilib>:"Write.vi"("Values"=w693, "DIO Ref In"=w689) -> ("DIO Ref Out"=w688:T15)  [unwired: 7 in, 1 out]
        n174 = node-c288(w716) -> ()  [unwired: 1 out]
      }
      n175 = timed-loop {
        shift-right: [w661] -> w93
        shift-left: 0 -> [w672]
        shift-right: [w662] -> _
        shift-left: 1 -> [w673]
        shift-right: [w658] -> _
        shift-left: 0 -> [w671]
        timing: w109 -> [_]
        timing-out: [_] -> w108
        tunnel: w65 -> [w648]
        tunnel: w64 -> [w647]
        tunnel: [w646] -> w84
        tunnel: [w645] -> w83
        tunnel: w52 -> [w643]
        stop <- w656 stop-if-true
        n176 = node-c288() -> ()  [unwired: 1 in, 1 out]
        n177 = call <vilib>:"Read.vi"("AI Ref In"=w643) -> ("Values"=w644:dbl[])  [unwired: 8 in, 2 out]
        n178 = Index Array(array=w644) -> (element=→"Optical Y":dbl)  [unwired: 1 in]
        n179 = control-ref of="Motor Input y"() -> (w665:refnum<vi>)
        n180 = control-ref of="User Input y"() -> (w664:refnum<vi>)
        n181 = control-ref of="Step diff y"() -> (w663:refnum<vi>)
        n182 = local read "Stop"() -> (w656:bool)
        n183 = call "Single Axis motor_Y(SubVI).vi"("State=1, I"=w673, "Motor=0, I"=w672, "Position=0, I"=w671, "User Input"="User Input y", "Motor Input"="Motor Input y", "Backward"="Left y", "Forward"="Right y", "Step diff"="Step diff y", "Motor input_L"=w665, "User input_L"=w664, "Step diff_L"=w663) -> ("right"=→"right y":bool, "down"=→"down y":bool, "Motor State"=→"Motor State y":dbl, "State=1, O"=w662:dbl, "Motor=0, O"=w661:i32, "Position=0, O"=w658:dbl, "Real Output"=→"Real Output y":dbl, "Motor Position"=→"Motor Position y":dbl, "up"=w650:bool, "left"=w649:bool, "Moving"=→"Moving y":bool)  [unwired: 5 in, 1 out]
        "up y" <- w650
        "left y" <- w649
        n184 = Reciprocal(x="Step/s y") -> (1/x=w676:dbl)
        n185 = Build Array(w650) -> (w652:bool[])
        n186 = Build Array(w649) -> (w651:bool[])
        n187 = call <vilib>:"Write.vi"("Values"=w652, "DIO Ref In"=w648) -> ("DIO Ref Out"=w645:T15)  [unwired: 7 in, 1 out]
        n188 = call <vilib>:"Write.vi"("Values"=w651, "DIO Ref In"=w647) -> ("DIO Ref Out"=w646:T15)  [unwired: 7 in, 1 out]
        n189 = Multiply(x=w676, y=1000) -> (x*y=w674:dbl)
        n190 = node-c288(w674) -> ()  [unwired: 1 out]
      }
      n191 = timed-loop {
        shift-right: [w619] -> w91
        shift-left: 0 -> [w630]
        shift-right: [w620] -> _
        shift-left: 1 -> [w631]
        shift-right: [w615] -> _
        shift-left: 0 -> [w629]
        timing: w101 -> [_]
        timing-out: [_] -> w100
        tunnel: w57 -> [w606]
        tunnel: w56 -> [w605]
        tunnel: [w604] -> w80
        tunnel: [w603] -> w79
        tunnel: w48 -> [w601]
        stop <- w613 stop-if-true
        n192 = node-c288() -> ()  [unwired: 1 in, 1 out]
        n193 = call <vilib>:"Read.vi"("AI Ref In"=w601) -> ("Values"=w602:dbl[])  [unwired: 8 in, 2 out]
        n194 = Index Array(array=w602) -> (element=→"Optical psi":dbl)  [unwired: 1 in]
        n195 = control-ref of="Motor Input psi"() -> (w623:refnum<vi>)
        n196 = control-ref of="User Input psi"() -> (w622:refnum<vi>)
        n197 = control-ref of="Step diff psi"() -> (w621:refnum<vi>)
        n198 = local read "Stop"() -> (w613:bool)
        n199 = call "Single Axis motor_Psi(SubVI).vi"("State=1, I"=w631, "Motor=0, I"=w630, "Position=0, I"=w629, "User Input"="User Input psi", "Motor Input"="Motor Input psi", "Backward"="Left psi", "Forward"="Right psi", "Step diff"="Step diff psi", "Motor input_L"=w623, "User input_L"=w622, "Step diff_L"=w621) -> ("right"=→"right psi":bool, "down"=→"down psi":bool, "Motor State"=→"Motor State psi":dbl, "State=1, O"=w620:dbl, "Motor=0, O"=w619:i32, "Position=0, O"=w615:dbl, "Real Output"=→"Real Output psi":dbl, "Motor Position"=→"Motor Position psi":dbl, "up"=w608:bool, "left"=w607:bool, "Moving"=→"Moving psi":bool)  [unwired: 5 in, 1 out]
        "up psi" <- w608
        "left psi" <- w607
        n200 = Reciprocal(x="Step/s psi") -> (1/x=w634:dbl)
        n201 = Build Array(w608) -> (w610:bool[])
        n202 = Build Array(w607) -> (w609:bool[])
        n203 = call <vilib>:"Write.vi"("Values"=w610, "DIO Ref In"=w606) -> ("DIO Ref Out"=w603:T15)  [unwired: 7 in, 1 out]
        n204 = call <vilib>:"Write.vi"("Values"=w609, "DIO Ref In"=w605) -> ("DIO Ref Out"=w604:T15)  [unwired: 7 in, 1 out]
        n205 = Multiply(x=w634, y=1000) -> (x*y=w632:dbl)
        n206 = node-c288(w632) -> ()  [unwired: 1 out]
      }
      n207 = timed-loop {
        shift-right: [w747] -> w92
        shift-left: 0 -> [w756]
        shift-right: [w748] -> _
        shift-left: 1 -> [w757]
        shift-right: [w743] -> _
        shift-left: 0 -> [w755]
        timing: w113 -> [_]
        timing-out: [_] -> w112
        tunnel: w61 -> [w732]
        tunnel: w60 -> [w731]
        tunnel: [w730] -> w82
        tunnel: [w729] -> w81
        tunnel: w50 -> [w727]
        stop <- w741 stop-if-true
        n208 = node-c288() -> ()  [unwired: 1 in, 1 out]
        n209 = call <vilib>:"Read.vi"("AI Ref In"=w727) -> ("Values"=w728:dbl[])  [unwired: 8 in, 2 out]
        n210 = Index Array(array=w728) -> (element=→"Optical Z":dbl)  [unwired: 1 in]
        n211 = control-ref of="Motor Input z"() -> (w751:refnum<vi>)
        n212 = control-ref of="User Input z"() -> (w750:refnum<vi>)
        n213 = control-ref of="Step diff z"() -> (w749:refnum<vi>)
        n214 = call "Single Axis motor_Z(SubVI).vi"("State=1, I"=w757, "Motor=0, I"=w756, "Position=0, I"=w755, "User Input"="User Input z", "Motor Input"="Motor Input z", "Backward"="Down z", "Forward"="Up z", "Step diff"="Step diff z", "Motor input_L"=w751, "User input_L"=w750, "Step diff_L"=w749) -> ("right"=→"right z":bool, "down"=→"down z":bool, "Motor State"=→"Motor State z":dbl, "State=1, O"=w748:dbl, "Motor=0, O"=w747:i32, "Position=0, O"=w743:dbl, "Real Output"=→"Real Output z":dbl, "Motor Position"=→"Motor Position z":dbl, "up"=w733:bool, "left"=w734:bool, "Moving"=→"Moving z":bool)  [unwired: 5 in, 1 out]
        "up z" <- w733
        "left z" <- w734
        n215 = local read "Stop"() -> (w741:bool)
        n216 = Reciprocal(x="Step/s z") -> (1/x=w760:dbl)
        n217 = Build Array(w733) -> (w736:bool[])
        n218 = Build Array(w734) -> (w735:bool[])
        n219 = call <vilib>:"Write.vi"("Values"=w736, "DIO Ref In"=w732) -> ("DIO Ref Out"=w729:T15)  [unwired: 7 in, 1 out]
        n220 = call <vilib>:"Write.vi"("Values"=w735, "DIO Ref In"=w731) -> ("DIO Ref Out"=w730:T15)  [unwired: 7 in, 1 out]
        n221 = Multiply(x=w760, y=1000) -> (x*y=w758:dbl)
        n222 = node-c288(w758) -> ()  [unwired: 1 out]
      }
      n223 = node-c288(w117) -> ()  [unwired: 1 out]
      n224 = node-c288(w110) -> ()  [unwired: 1 out]
      n225 = node-c288(w108) -> ()  [unwired: 1 out]
      n226 = node-c288(w100) -> ()  [unwired: 1 out]
      n227 = node-c288(w112) -> ()  [unwired: 1 out]
      n228 = while {
        tunnel: w31 -> [w121]
        tunnel: [w120] -> w32
        shift-right: [w122] -> w33
        shift-left: w30 -> [w119]
        stop <- w123 stop-if-true
        # "TCP Write Loop"
        n229 = case shown="No Error" w119 {
          tunnel: [w128 w151] -> w122
          tunnel: w121 -> [w127 w152]
          tunnel: [w126 w152] -> w120
          tunnel: w119 -> [w125 w151]
          frame No Error {
            n230 = local read "Moving x"() -> (w135:bool)
            n231 = local read "Real Output x"() -> (w137:dbl)
            n232 = local read "Moving y"() -> (w138:bool)
            n233 = local read "Real Output y"() -> (w140:dbl)
            n234 = local read "Moving z"() -> (w142:bool)
            n235 = local read "Real Output z"() -> (w144:dbl)
            n236 = local read "Moving psi"() -> (w141:bool)
            n237 = local read "Real Output psi"() -> (w146:dbl)
            n238 = local read "Moving"() -> (w147:bool)
            n239 = local read "Real Output theta"() -> (w149:dbl)
            n240 = local read "Real Output Phi"() -> (w150:dbl)
            n241 = Boolean To (0,1)(Boolean=w135) -> (0, 1=w136:i16)
            n242 = Boolean To (0,1)(Boolean=w138) -> (0, 1=w139:i16)
            n243 = Boolean To (0,1)(Boolean=w142) -> (0, 1=w143:i16)
            n244 = Boolean To (0,1)(Boolean=w147) -> (0, 1=w148:i16)
            n245 = Boolean To (0,1)(Boolean=w141) -> (0, 1=w145:i16)
            n246 = Build Array(w136, w137, w139, w140, w143, w144, w145, w146, w148, w149, w150) -> (w134:dbl[])
            n247 = To Single Precision Float(number=w134) -> (single precision float=w133:sgl[])
            n248 = Flatten To String(anything=w133, prepend array or string size? (T)=FALSE, byte order (0:big-endian, network order)=T1."big-endian, network order") -> (data string=w132:string)  [unwired: 1 in, 2 out]
            n249 = TCP Write(connection ID=w127, data in=w132, error in (no error)=w125, 9:1000) -> (connection ID out=w126:refnum<k5>, error out=w128:errorcluster)  [unwired: 1 out]
          }
          frame Error {
          }
        }
        n250 = Wait (ms)(milliseconds to wait=100) -> ()  [unwired: 1 out]
        n251 = local read "Stop"() -> (w123:bool)
      }
    }
    frame #2 {
      n252 = TCP Close Connection(connection ID=w846, error in (no error)=w847) -> ()  [unwired: 3 out]
      n253 = node-c288() -> (w874:T4)  [unwired: 4 in]
      n254 = node-c288() -> (w877:T4)  [unwired: 4 in]
      n255 = node-c288() -> (w880:T4)  [unwired: 4 in]
      n256 = node-c288() -> (w883:T4)  [unwired: 4 in]
      n257 = node-c288() -> (w886:T4)  [unwired: 4 in]
      n258 = node-c288() -> (w889:T4)  [unwired: 4 in]
      n259 = timed-loop {
        timing: w874 -> [_]
        timing-out: [_] -> w873
        shift-right: [w899] -> _
        shift-left: w872 -> [w903]
        tunnel: w872 -> [w904]
        tunnel: w855 -> [w893]
        tunnel: w854 -> [w892]
        tunnel: [w891] -> w849
        tunnel: [w890] -> w848
        i -> [w902]
        stop <- w898 stop-if-true
        n260 = node-c288() -> ()  [unwired: 1 in, 1 out]
        n261 = control-ref of="Stop number psi"() -> (w900:refnum<vi>)
        n262 = call "Motor stop_Psi(SubVI).vi"("Motor, C"=w904, "Motor, I"=w903, "i"=w902, "Stop number"="Stop number psi", "Stop number_L"=w900) -> ("Motor, O"=w899:i32, "Loop stop"=w898:bool, "up"=w895:bool, "left"=w894:bool)  [unwired: 7 in]
        n263 = Build Array(w895) -> (w896:bool[])
        n264 = Build Array(w894) -> (w897:bool[])
        n265 = call <vilib>:"Write.vi"("Values"=w896, "DIO Ref In"=w892) -> ("DIO Ref Out"=w891:T15)  [unwired: 7 in, 1 out]
        n266 = call <vilib>:"Write.vi"("Values"=w897, "DIO Ref In"=w893) -> ("DIO Ref Out"=w890:T15)  [unwired: 7 in, 1 out]
        n267 = node-c288(100) -> ()  [unwired: 1 out]
      }
      n268 = timed-loop {
        timing: w877 -> [_]
        timing-out: [_] -> w876
        shift-right: [w921] -> _
        shift-left: w875 -> [w925]
        tunnel: w875 -> [w926]
        tunnel: w857 -> [w914]
        tunnel: w856 -> [w915]
        tunnel: [w913] -> w851
        tunnel: [w912] -> w850
        i -> [w924]
        stop <- w920 stop-if-true
        n269 = node-c288() -> ()  [unwired: 1 in, 1 out]
        n270 = control-ref of="Stop number z"() -> (w922:refnum<vi>)
        n271 = call "Motor stop_Z(SubVI).vi"("Motor, C"=w926, "Motor, I"=w925, "i"=w924, "Stop number"="Stop number z", "Stop number_L"=w922) -> ("Motor, O"=w921:i32, "Loop stop"=w920:bool, "up"=w917:bool, "left"=w916:bool)  [unwired: 7 in]
        n272 = Build Array(w917) -> (w918:bool[])
        n273 = Build Array(w916) -> (w919:bool[])
        n274 = call <vilib>:"Write.vi"("Values"=w918, "DIO Ref In"=w915) -> ("DIO Ref Out"=w913:T15)  [unwired: 7 in, 1 out]
        n275 = call <vilib>:"Write.vi"("Values"=w919, "DIO Ref In"=w914) -> ("DIO Ref Out"=w912:T15)  [unwired: 7 in, 1 out]
        n276 = node-c288(100) -> ()  [unwired: 1 out]
      }
      n277 = timed-loop {
        timing: w880 -> [_]
        timing-out: [_] -> w879
        shift-right: [w943] -> _
        shift-left: w878 -> [w947]
        tunnel: w878 -> [w948]
        tunnel: w859 -> [w937]
        tunnel: w858 -> [w936]
        tunnel: [w935] -> w853
        tunnel: [w934] -> w852
        i -> [w946]
        stop <- w942 stop-if-true
        n278 = node-c288() -> ()  [unwired: 1 in, 1 out]
        n279 = control-ref of="Stop number y"() -> (w944:refnum<vi>)
        n280 = call "Motor stop_Y(SubVI).vi"("Motor, C"=w948, "Motor, I"=w947, "i"=w946, "Stop number"="Stop number y", "Stop number_L"=w944) -> ("Motor, O"=w943:i32, "Loop stop"=w942:bool, "up"=w939:bool, "left"=w938:bool)  [unwired: 7 in]
        n281 = Build Array(w939) -> (w940:bool[])
        n282 = Build Array(w938) -> (w941:bool[])
        n283 = call <vilib>:"Write.vi"("Values"=w940, "DIO Ref In"=w936) -> ("DIO Ref Out"=w935:T15)  [unwired: 7 in, 1 out]
        n284 = call <vilib>:"Write.vi"("Values"=w941, "DIO Ref In"=w937) -> ("DIO Ref Out"=w934:T15)  [unwired: 7 in, 1 out]
        n285 = node-c288(100) -> ()  [unwired: 1 out]
      }
      n286 = timed-loop {
        timing: w883 -> [_]
        timing-out: [_] -> w882
        shift-right: [w965] -> _
        shift-left: w881 -> [w969]
        tunnel: w881 -> [w970]
        tunnel: [w959] -> w863
        tunnel: [w958] -> w862
        tunnel: w861 -> [w957]
        tunnel: w860 -> [w956]
        i -> [w968]
        stop <- w964 stop-if-true
        n287 = node-c288() -> ()  [unwired: 1 in, 1 out]
        n288 = control-ref of="Stop number x"() -> (w966:refnum<vi>)
        n289 = call "Motor stop_X(SubVI).vi"("Motor, C"=w970, "Motor, I"=w969, "i"=w968, "Stop number"="Stop number x", "Stop number_L"=w966) -> ("Motor, O"=w965:i32, "Loop stop"=w964:bool, "up"=w961:bool, "left"=w960:bool)  [unwired: 7 in]
        n290 = Build Array(w961) -> (w962:bool[])
        n291 = Build Array(w960) -> (w963:bool[])
        n292 = call <vilib>:"Write.vi"("Values"=w962, "DIO Ref In"=w956) -> ("DIO Ref Out"=w959:T15)  [unwired: 7 in, 1 out]
        n293 = call <vilib>:"Write.vi"("Values"=w963, "DIO Ref In"=w957) -> ("DIO Ref Out"=w958:T15)  [unwired: 7 in, 1 out]
        n294 = node-c288(100) -> ()  [unwired: 1 out]
      }
      n295 = timed-loop {
        timing: w886 -> [_]
        timing-out: [_] -> w885
        shift-right: [w987] -> _
        shift-left: w884 -> [w991]
        tunnel: w884 -> [w992]
        tunnel: w867 -> [w981]
        tunnel: w866 -> [w980]
        tunnel: [w979] -> w865
        tunnel: [w978] -> w864
        i -> [w990]
        stop <- w986 stop-if-true
        n296 = node-c288() -> ()  [unwired: 1 in, 1 out]
        n297 = control-ref of="Stop number R"() -> (w988:refnum<vi>)
        n298 = call "Motor stop_R(SubVI).vi"("Motor, C"=w992, "Motor, I"=w991, "i"=w990, "Stop number"="Stop number R", "Stop number_L"=w988) -> ("Motor, O"=w987:i32, "Loop stop"=w986:bool, "up"=w983:bool, "left"=w982:bool)  [unwired: 7 in]
        n299 = Build Array(w983) -> (w984:bool[])
        n300 = Build Array(w982) -> (w985:bool[])
        n301 = call <vilib>:"Write.vi"("Values"=w984, "DIO Ref In"=w981) -> ("DIO Ref Out"=w979:T15)  [unwired: 7 in, 1 out]
        n302 = call <vilib>:"Write.vi"("Values"=w985, "DIO Ref In"=w980) -> ("DIO Ref Out"=w978:T15)  [unwired: 7 in, 1 out]
        n303 = node-c288(100) -> ()  [unwired: 1 out]
      }
      n304 = timed-loop {
        timing: w889 -> [_]
        timing-out: [_] -> w888
        shift-right: [w1009] -> _
        shift-left: w887 -> [w1013]
        tunnel: w887 -> [w1014]
        tunnel: [w1003] -> w871
        tunnel: [w1002] -> w870
        tunnel: w869 -> [w1001]
        tunnel: w868 -> [w1000]
        i -> [w1012]
        stop <- w1008 stop-if-true
        n305 = node-c288() -> ()  [unwired: 1 in, 1 out]
        n306 = control-ref of="Stop number L"() -> (w1010:refnum<vi>)
        n307 = call "Motor stop_L(SubVI).vi"("Motor, C"=w1014, "Motor, I"=w1013, "i"=w1012, "Stop number"="Stop number L", "Stop number_L"=w1010) -> ("Motor, O"=w1009:i32, "Loop stop"=w1008:bool, "up"=w1005:bool, "left"=w1004:bool)  [unwired: 7 in]
        n308 = Build Array(w1005) -> (w1006:bool[])
        n309 = Build Array(w1004) -> (w1007:bool[])
        n310 = call <vilib>:"Write.vi"("Values"=w1006, "DIO Ref In"=w1001) -> ("DIO Ref Out"=w1003:T15)  [unwired: 7 in, 1 out]
        n311 = call <vilib>:"Write.vi"("Values"=w1007, "DIO Ref In"=w1000) -> ("DIO Ref Out"=w1002:T15)  [unwired: 7 in, 1 out]
        n312 = node-c288(100) -> ()  [unwired: 1 out]
      }
      n313 = node-c288(w873) -> ()  [unwired: 1 out]
      n314 = node-c288(w876) -> ()  [unwired: 1 out]
      n315 = node-c288(w879) -> ()  [unwired: 1 out]
      n316 = call <vilib>:"Close.vi"("DIO Ref In"=w849) -> ()  [unwired: 10 in, 1 out]
      n317 = call <vilib>:"Close.vi"("DIO Ref In"=w848) -> ()  [unwired: 10 in, 1 out]
      n318 = node-c288(w882) -> ()  [unwired: 1 out]
      n319 = call <vilib>:"Close.vi"("DIO Ref In"=w851) -> ()  [unwired: 10 in, 1 out]
      n320 = call <vilib>:"Close.vi"("DIO Ref In"=w850) -> ()  [unwired: 10 in, 1 out]
      n321 = node-c288(w885) -> ()  [unwired: 1 out]
      n322 = call <vilib>:"Close.vi"("DIO Ref In"=w853) -> ()  [unwired: 10 in, 1 out]
      n323 = node-c288(w888) -> ()  [unwired: 1 out]
      n324 = call <vilib>:"Close.vi"("DIO Ref In"=w852) -> ()  [unwired: 10 in, 1 out]
      n325 = call <vilib>:"Close.vi"("DIO Ref In"=w863) -> ()  [unwired: 10 in, 1 out]
      n326 = call <vilib>:"Close.vi"("DIO Ref In"=w862) -> ()  [unwired: 10 in, 1 out]
      n327 = call <vilib>:"Close.vi"("DIO Ref In"=w871) -> ()  [unwired: 10 in, 1 out]
      n328 = call <vilib>:"Close.vi"("DIO Ref In"=w870) -> ()  [unwired: 10 in, 1 out]
      n329 = call <vilib>:"Close.vi"("DIO Ref In"=w865) -> ()  [unwired: 10 in, 1 out]
      n330 = call <vilib>:"Close.vi"("DIO Ref In"=w864) -> ()  [unwired: 10 in, 1 out]
    }
  }
